vi "set Attenuation.vi"(8 "error in (no error)":errorcluster, 9 "Auto?":bool, 10 "Attenuation":i32, 11 "FSV-40N in":refnum<class "FSV-40N.lvclass">) -> (0 "error out":errorcluster, 3 "FSV-40N out":refnum<class "FSV-40N.lvclass">)   [LabVIEW 2023, in "Spectrum Analyzer.lvlib" / "FSV-40N.lvclass"]
uses:
  FSV-40N.lvclass
  FSV-40N.lvclass/FSV-40N.ctl
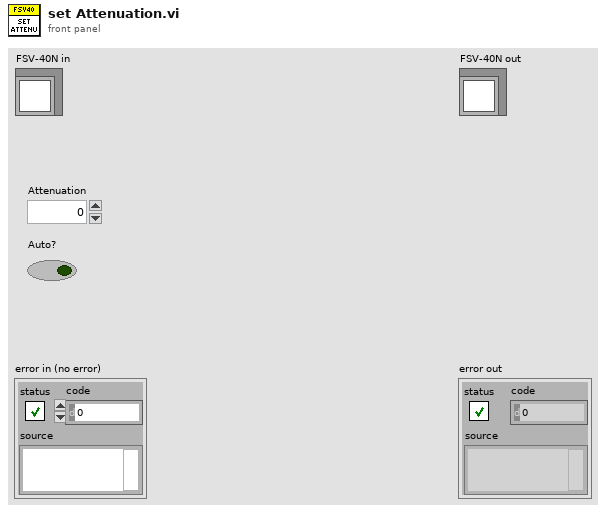
[diagram p1: front panel]
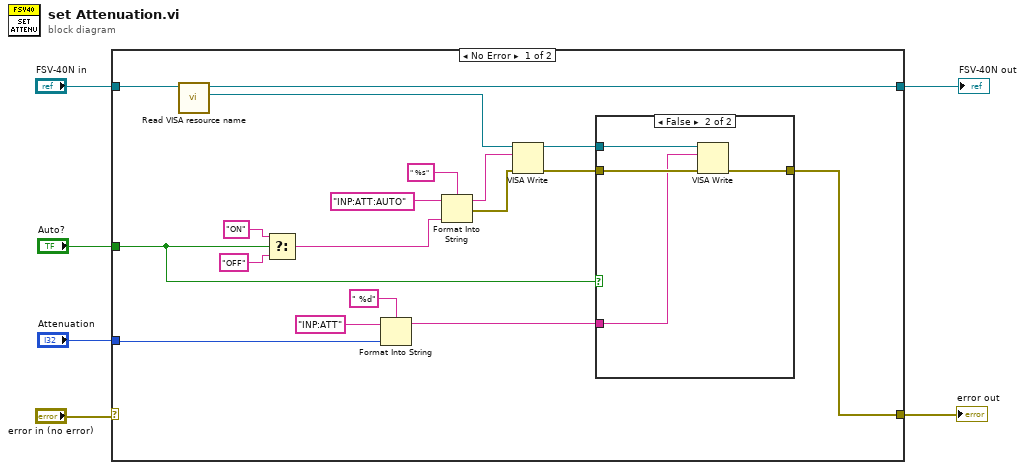
[diagram p0: block diagram]
diagram:
  n1 = case shown="No Error" "error in (no error)" {
    selector: "error in (no error)" -> [_ w30]
    tunnel: "FSV-40N in" -> [w24 w31]
    tunnel: [w23 w31] -> w3
    tunnel: [w22 w30] -> w2
    tunnel: "Auto?" -> [w8 _]
    tunnel: "Attenuation" -> [w12 _]
    frame No Error {
      n2 = call "Read VISA resource name.vi"("FSV-40N in"=w24) -> ("VISA resource name"=w16:refnum<visa-resource-name>, "FSV-40N out"=w23:refnum<class "FSV-40N.lvclass">)  [unwired: 8 in, 1 out]
      n3 = Select(t="ON", s=w8, f="OFF") -> (s? t:f=w17:string)
      n4 = Format Into String(format string=" %d", initial string="INP:ATT" ("write buffer"), w12) -> (resulting string=w7:string)  [unwired: 1 in, 1 out]
      n5 = Format Into String(format string=" %s", initial string="INP:ATT:AUTO" ("write buffer"), w17) -> (resulting string=w15:string, error out=w14:errorcluster)  [unwired: 1 in]
      n6 = VISA Write(VISA resource name=w16, write buffer=w15, error in (no error)=w14) -> (VISA resource name out=w10:refnum<visa-resource-name>, error out=w9:errorcluster)  [unwired: 1 out]
      n7 = case shown="False" w8 {
        tunnel: w10 -> [_ w29]
        tunnel: [w25 w28] -> w22
        tunnel: w9 -> [w25 w27]
        tunnel: w7 -> [_ w26]
        frame True {
        }
        frame False {
          n8 = VISA Write(VISA resource name=w29, write buffer=w26, error in (no error)=w27) -> (error out=w28:errorcluster)  [unwired: 2 out]
        }
      }
    }
    frame Error {
    }
  }
  "error out" <- w2
  "FSV-40N out" <- w3
